vi "connection.create_connection.vi"(7 "description":string, 8 "error in":errorcluster, 9 "nominalDataSourceRid":string, 10 "name":string, 11 "Nominal Client in":refnum<class "Nominal Client.lvclass">) -> (0 "error out":errorcluster, 1 "Response":string, 2 "response":T1, 3 "Nominal Client out":refnum<class "Nominal Client.lvclass">)   [LabVIEW 2020, in "Nominal Client.lvclass"]
doc: "Creates a new connection.\n\nIf the ID is not unique, a timestamp will be added to the ID."
uses:
  Nominal Client.lvclass
  301638a4-f299-4835-8683-15cfc56d6fd6.vi
  <vilib>/JDP Science/JSONtext/JSONtext.lvlib
  28804fc9-aee6-4b6e-ba11-1ba961eefadd.vi
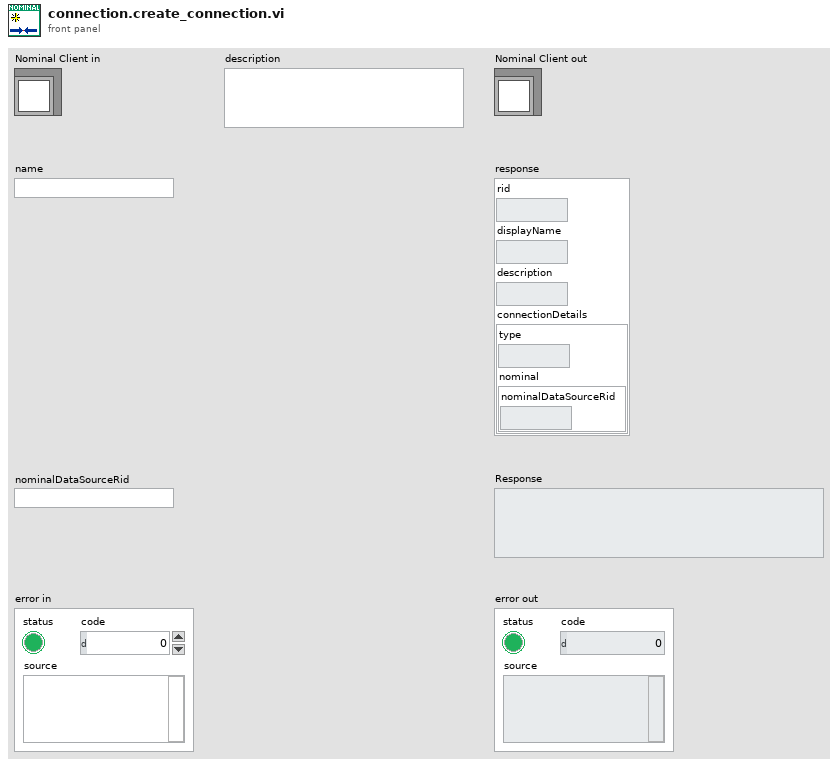
[diagram p1: front panel]
types:
  T1 = cluster{"rid":string, "displayName":string, "description":string, "connectionDetails":cluster{"type":string, "nominal":cluster{"nominalDataSourceRid":string}}}
  T2 = cluster{"type":string, "nominal":cluster{"nominalDataSourceRid":string}}
  T3 = cluster{"name":string, "description":string, "connectionDetails":cluster{"type":string, "nominal":cluster{"nominalDataSourceRid":string}}}
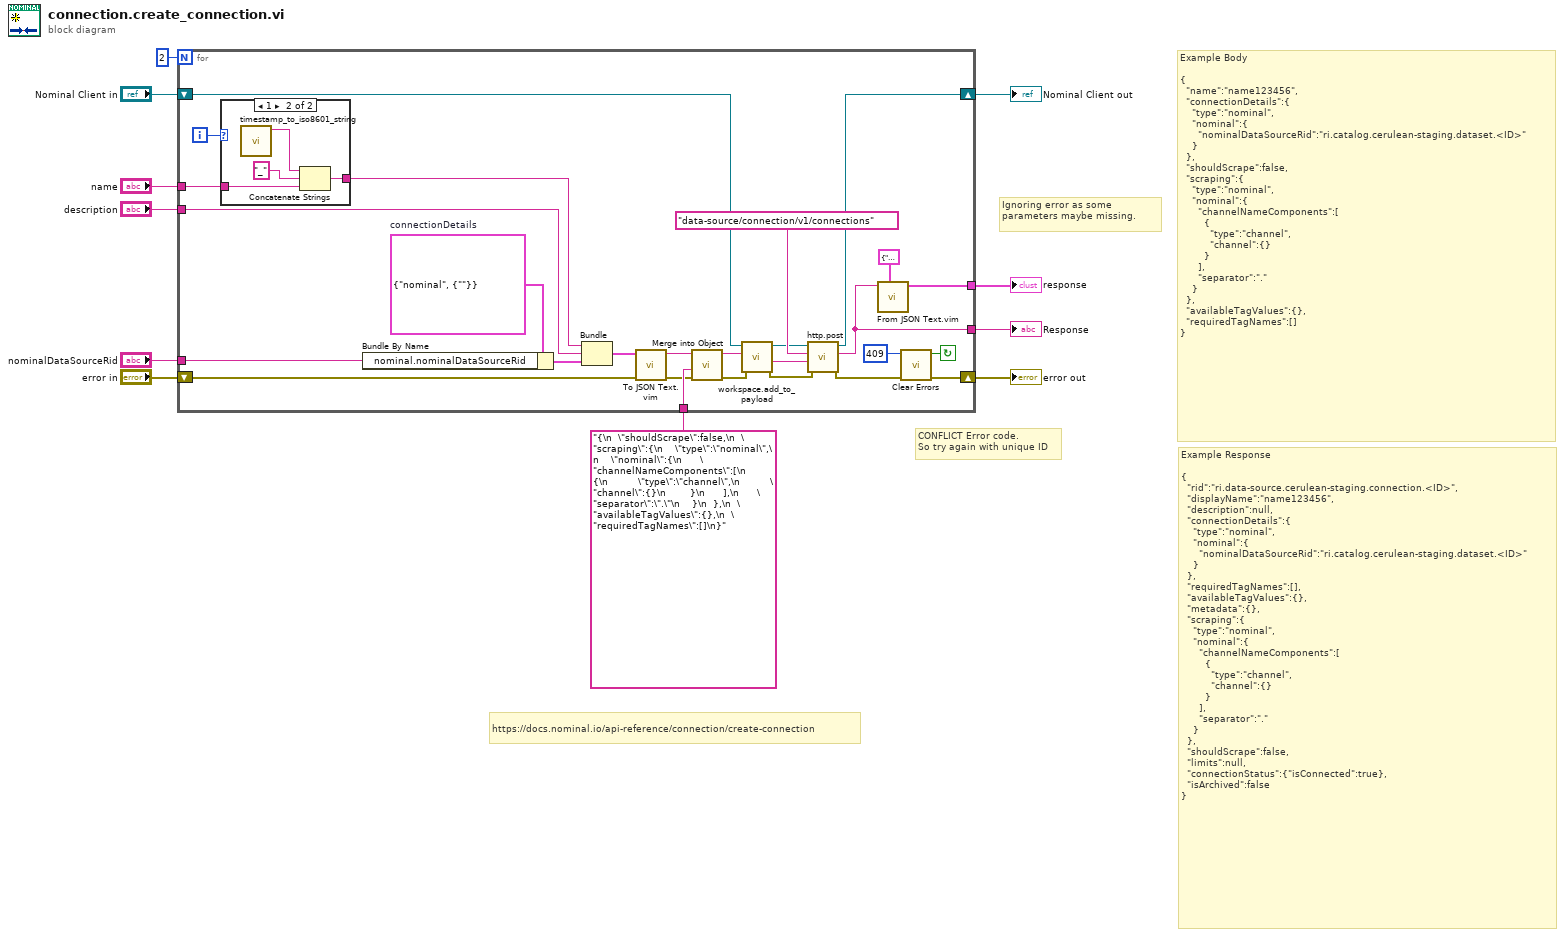
[diagram p0: block diagram]
diagram:
  # "CONFLICT Error code.\nSo try again with unique ID"
  # "https://docs.nominal.io/api-reference/connection/create-connection"
  # "Ignoring error as some parameters maybe missing."
  # "Example Response\n\n{\n  \"rid\":\"ri.data-source.cerulean-staging.connection.<ID>\",\n  \"displayName\":\"name123456\",\n  \"description\":null,\n  \"connectionDetails\":{\n    \"type\":\"nominal\",\n    \"nominal\":{\n      \"nominalDataSourceRid\":\"ri.catalog.cerulean-staging.dataset.<ID>\"\n    }\n  },\n  \"requiredTagNames\":[],\n  \"availableTagValues\":{},\n  \"metadata\":{},\n  \"scraping\":{\n    \"type\":\"nominal\",\n    \"nominal\":{\n      \"channelNameComponents\":[\n        {\n          \"type\":\"channel\",\n          \"channel\":{}\n        }\n      ],\n      \"separator\":\".\"\n    }\n  },\n  \"shouldScrape\":false,\n  \"limits\":null,\n  \"connectionStatus\":{\"isConnected\":true},\n  \"isArchived\":false\n}"
  # "Example Body\n\n{\n  \"name\":\"name123456\",\n  \"connectionDetails\":{\n    \"type\":\"nominal\",\n    \"nominal\":{\n      \"nominalDataSourceRid\":\"ri.catalog.cerulean-staging.dataset.<ID>\"\n    }\n  },\n  \"shouldScrape\":false,\n  \"scraping\":{\n    \"type\":\"nominal\",\n    \"nominal\":{\n      \"channelNameComponents\":[\n        {\n          \"type\":\"channel\",\n          \"channel\":{}\n        }\n      ],\n      \"separator\":\".\"\n    }\n  },\n  \"availableTagValues\":{},\n  \"requiredTagNames\":[]\n}"
  n1 = for {
    N: 2 -> [_]
    tunnel: "nominalDataSourceRid" -> [w36]
    tunnel: [w26] -> w4
    tunnel: "name" -> [w19]
    tunnel: "description" -> [w25]
    shift-right: [w32] -> w7
    shift-left: "Nominal Client in" -> [w13]
    shift-right: [w22] -> w8
    shift-left: "error in" -> [w34]
    tunnel: "{\n  \"shouldScrape\":false,\n  \"scraping\":{\n    \"type\":\"nominal\",\n    \"nominal\":{\n      \"channelNameComponents\":[\n        {\n          \"type\":\"channel\",\n          \"channel\":{}\n        }\n      ],\n      \"separator\":\".\"\n    }\n  },\n  \"availableTagValues\":{},\n  \"requiredTagNames\":[]\n}" ("Request body") -> [w31]
    tunnel: [w28] -> w5
    i -> [w20]
    stop <- w24 continue-if-true
    w38 = T2 {"type"="nominal", "nominal"={"nominalDataSourceRid"=""}}  # connectionDetails
    n2 = case shown="1" w20 {
      tunnel: w19 -> [w39 w43]
      tunnel: [w39 w42] -> w18
      frame 0, Default {
      }
      frame 1 {
        n3 = call "timestamp_to_iso8601_string.vi"() -> ("ISO8601 UTC DateTime"=w40:string)  [unwired: 11 in]
        n4 = Concatenate Strings(w40, "_" ("string"), w43) -> (w42:string)
      }
    }
    n5 = Bundle By Name(cluster=w38, "nominal.nominalDataSourceRid"=w36) -> (w37:T2)
    n6 = Bundle("name"=w18, "description"=w25, "connectionDetails"=w37) -> (w35:T3)  [unwired: 1 in]
    n7 = call "To JSON Text.vim"("error in (no error)"=w34, "Anything"=w35) -> ("error out"=w29:errorcluster, "<JSON>"=w30:string)  [unwired: 8 in]
    n8 = call <vilib>:"Merge into Object.vi"("error in (no error)"=w29, "JSON Object to Merge"=w31, "JSON"=w30) -> ("error out"=w15:errorcluster, "<JSON>"=w17:string)  [unwired: 6 in]
    n9 = call "workspace.add_to_payload.vi"("error in"=w15, "JSON payload in"=w17, "Nominal Client in"=w13) -> ("error out"=w16:errorcluster, "JSON payload out"=w12:string, "Nominal Client out"=w14:refnum<class "Nominal Client.lvclass">)  [unwired: 6 in]
    n10 = call "http.post.vi"("error in"=w16, "Request body"=w12, "Path"="data-source/connection/v1/connections", "Nominal Client in"=w14) -> ("error out"=w23:errorcluster, "Response"=w28:string, "Nominal Client out"=w32:refnum<class "Nominal Client.lvclass">)  [unwired: 4 in, 1 out]
    n11 = call "From JSON Text.vim"("Data Type and Default Value"=T1 {"rid"="", "displayName"="", "description"="", "connectionDetails"={"type"="", "nominal"={"nominalDataSourceRid"=""}}} ("response"), "JSON"=w28) -> ("Data out"=w26:T1)  [unwired: 8 in, 1 out]
    n12 = call <vilib>:"Clear Errors.vi"("error in (no error)"=w23, "specific error code to clear (0: all)"=409) -> ("error out"=w22:errorcluster, "specific error cleared?"=w24:bool)  [unwired: 4 in]
  }
  "Nominal Client out" <- w7
  "error out" <- w8
  "Response" <- w5
  "response" <- w4
